vi "AdaptToInputs.vi"(3 "Term Types":T1, 4 "XRef":refnum<vi>, 5 "State In":T5) -> (0 "Reply":string[](array[string]), 2 "State Out":T5)   [LabVIEW 2012, in "OpenG Index Array Element.xnode"]
uses:
  OpenG Index Array Element.xnode
  State.ctl
  <vilib>/XNodeSupport/XNodeTermTypeIDPairs.ctl
  <vilib>/XNodeSupport/XNodeTermTypeIDPair.ctl
  <vilib>/XNodeSupport/XNodeType.ctl
  <vilib>/XNodeSupport/XNodeString.ctl
  <userlib>/_LAVAcr/Scripting Tools/XNode Support/TypeDefs/Array Dimension Tests.ctl
  <userlib>/_LAVAcr/Scripting Tools/XNode Support/Find term type by ID_type.vi
  <userlib>/_LAVAcr/Scripting Tools/XNode Support/XNode Support.lvlib
  <vilib>/XNodeSupport/NI_XNodeSupport.lvlib
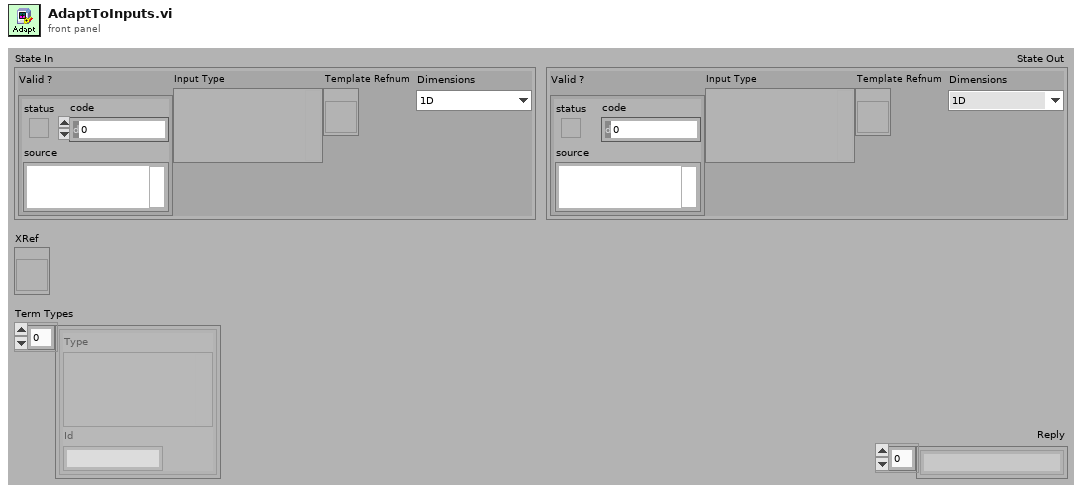
[diagram p1: front panel]
types:
  T1 = typedef "NI_XNodeSupport.lvlib/XNodeTermTypeIDPairs.ctl" = T2[]
  T2 = typedef "NI_XNodeSupport.lvlib/XNodeTermTypeIDPair.ctl" = cluster{"Type":T3, "Id":T4}
  T3 = typedef "NI_XNodeSupport.lvlib/XNodeType.ctl" = variant
  T4 = typedef "NI_XNodeSupport.lvlib/XNodeString.ctl" = string
  T5 = typedef "OpenG Index Array Element.xnode/State.ctl" = cluster{"Valid ?":errorcluster, "Input Type":variant, "Template Refnum":refnum<vi>, "Dimensions":enum16{"1D", "2D"}}
  T6 = typedef "Scripting Tools.lvlib/XNode Support.lvlib/Array Dimension Tests.ctl" = enum16{"No Check", "At Least n dimensions", "Exactly N Dimensions", "No More Than N Dimensions"}
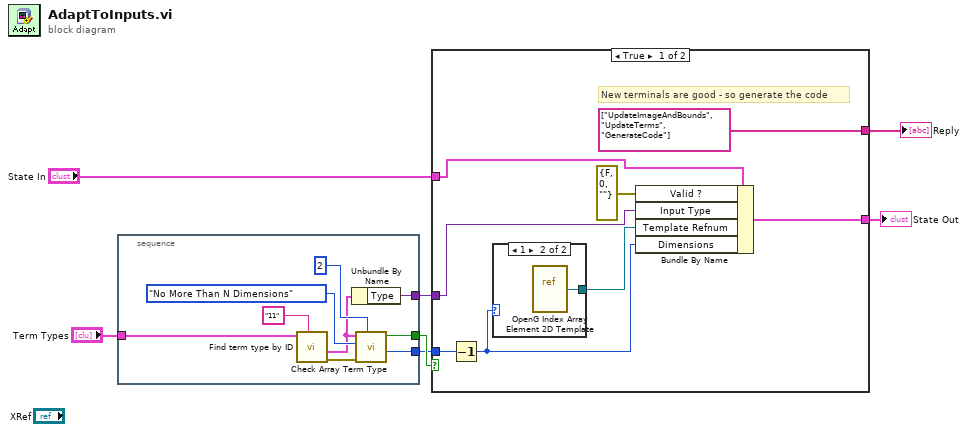
[diagram p0: block diagram]
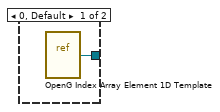
[diagram p2: hidden frame]
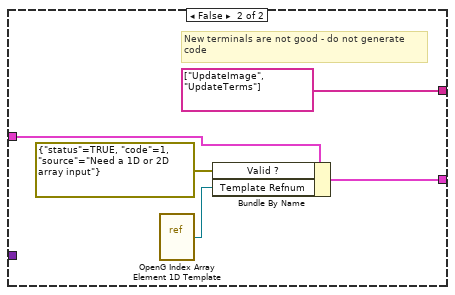
[diagram p3: hidden frame]
diagram:
  n1 = stacked-sequence {
    tunnel: "Term Types" -> [w16]
    tunnel: [w11] -> w6
    tunnel: [w8] -> w2
    tunnel: [w10] -> w1
    frame #0 {
      n2 = call-poly <userlib>:"Find term type by ID.vi"("Search ID"="11", "Term Types"=w16) -> ("error out"=w14:errorcluster, "Term Type"=w9:T2)  [unwired: 1 in, 7 out]
      n3 = Unbundle By Name(w9) -> ("Type"=w8:T3)
      n4 = call <userlib>:"Check Array Term Type.vi"("Dimensions Required"=2, "error in (no error)"=w14, "Dimension Check"=Array_Dimension_Tests."No More Than N Dimensions", "Term Type"=w9) -> ("Array Dimensions"=w10:i32, "Is Good ?"=w11:bool)  [unwired: 1 in, 5 out]
    }
  }
  n5 = case shown="True" w6 {
    tunnel: "State In" -> [w24 w31]
    tunnel: [w22 w29] -> w4
    tunnel: [string[] ["UpdateImageAndBounds", "UpdateTerms", "GenerateCode"] ("Reply") string[] ["UpdateImage", "UpdateTerms"] ("Reply")] -> w3
    tunnel: w2 -> [w19 _]
    tunnel: w1 -> [w18 _]
    frame True {
      # "New terminals are good - so generate the code"
      n6 = Decrement(x=w18) -> (x-1=w17:i32)
      n7 = case shown="1" w17 {
        tunnel: [w25 w26] -> w20
        frame 0, Default {
          n8 = vi-ref "OpenG Index Array Element 1D Template.vi"() -> (w25:refnum<vi>)
        }
        frame 1 {
          n9 = vi-ref "OpenG Index Array Element 2D Template.vi"() -> (w26:refnum<vi>)
        }
      }
      n10 = Bundle By Name(cluster=w24, "Valid ?"=errorcluster {"status"=FALSE, "code"=0, "source"=""}, "Input Type"=w19, "Template Refnum"=w20, "Dimensions"=w17) -> (w22:T5)
    }
    frame False {
      # "New terminals are not good - do not generate\ncode"
      n11 = vi-ref "OpenG Index Array Element 1D Template.vi"() -> (w27:refnum<vi>)
      n12 = Bundle By Name(cluster=w31, "Valid ?"=errorcluster {"status"=TRUE, "code"=1, "source"="Need a 1D or 2D array input"}, "Template Refnum"=w27) -> (w29:T5)
    }
  }
  "Reply" <- w3
  "State Out" <- w4
